vi "Own20261012_GetPropertyInfo.vi"() -> ()   [LabVIEW 2024]
uses:
  <vilib>/_script/All Supported PropertiesOrMethods TypeDefs/ASPM_UniqueIDStringDatanameShortnameLongname.ctl
  <vilib>/_script/All Supported PropertiesOrMethods TypeDefs/ASPM_ArrayOfUniqueIDStringDatanameShortnameLongname.ctl
panel:
  out "error out":errorcluster caption="错误输出"
  out "properties":T1 caption="属性[]"
  out "property_item_ids":refnum<vi>[](array[refnum])
  out "property_count":i32
  out "supported_properties":T1 caption="全部支持属性"
  out "class_name":string
  in  "property_id":u32
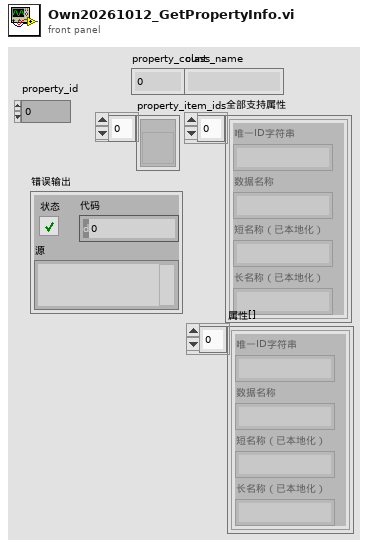
[diagram p1: front panel]
types:
  T1 = typedef "ASPM_ArrayOfUniqueIDStringDatanameShortnameLongname.ctl" = T2[]
  T2 = typedef "ASPM_UniqueIDStringDatanameShortnameLongname.ctl" = cluster{"Unique ID string":string, "Data name":string, "Short name (localized)":string, "Long name (localized)":string}
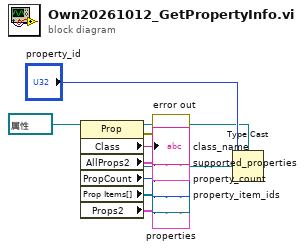
[diagram p0: block diagram]
diagram:
  n1 = Type Cast(type=refnum<vi> refnum ("引用"), x="property_id") -> (*(type *) &x=w7:refnum<vi>)
  n2 = property class="Prop"(reference=w7) -> (error out=→"error out":errorcluster, "Class"=→"class_name":string, "AllProps2"=→"supported_properties":T1, "PropCount"=→"property_count":i32, "Prop Items[]"=→"property_item_ids":refnum<vi>[], "Props2"=→"properties":T1)  [unwired: 1 in, 1 out]
